vi "PR_CTICA3_PARTE_C.vi"() -> ()   [LabVIEW 2026]
panel:
  in  "Tab Control":T1(tab)
  in  "Fila":dbl
  out "Modificado":dbl[][](array[numeric])
  in  "Fila Nueva":dbl[](array[numeric])
  in  "Columna Nueva":dbl[](array[numeric])
  out "Modificado  2":dbl[][](array[numeric])
  in  "Originales":dbl[][](array[numeric])
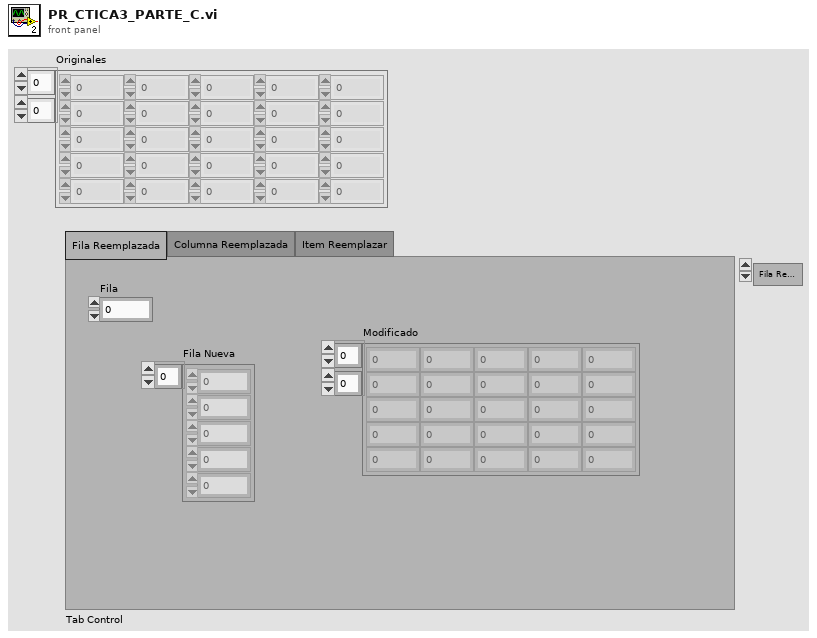
[diagram p1: front panel]
types:
  T1 = enum32{"Fila Reemplazada", "Columna Reemplazada", "Item Reemplazar"}
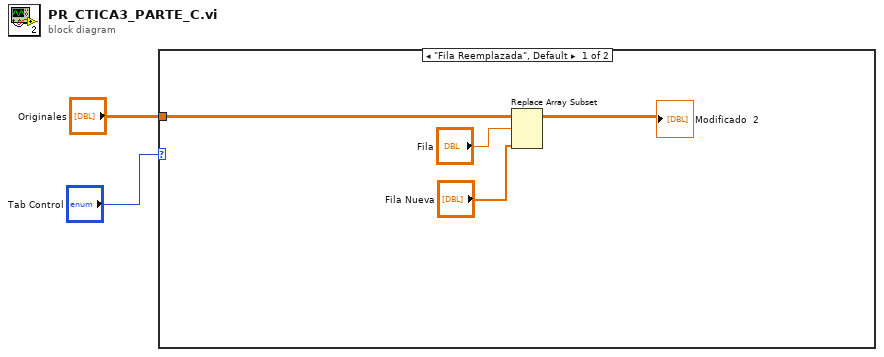
[diagram p0: block diagram]
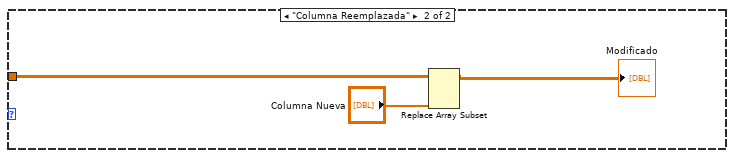
[diagram p2: hidden frame]
diagram:
  n1 = case shown="\"Fila Reemplazada\", Default" "Tab Control" {
    tunnel: "Originales" -> [w6 w9]
    frame "Fila Reemplazada", Default {
      n2 = Replace Array Subset(array=w6, new element="Fila Nueva", index (row)="Fila") -> (→"Modificado  2":dbl[][])  [unwired: 1 in]
    }
    frame "Columna Reemplazada" {
      n3 = Replace Array Subset(array=w9, new element="Columna Nueva") -> (→"Modificado":dbl[][])  [unwired: 2 in]
    }
  }
